vi "CE Center - VC manager.vi"(5 "cmd":enum16{"open", "close", "close all"}(ring)=enum."close", 6 "error in":errorcluster, 9 "VC Handle":T2=-1) -> (0 "error out":errorcluster, 1 "err code":T1 items=["No error", "Invalid variable type", "Variable not found", "Variable already exists", "Invalid context handle", "Input error", "Invalid data format", "No history attached", "History already attached", "Invalid history parameters", "Wrong variable name", "Wrong alias name", "Non-unique alias", "Alias not found", "No alias associated", "Alias already associated", "Wrong context name", "Non-unique context name", "Context name not found", "Invalid parameter", "Generic error", "Unknown error code"], 3 "VC Handle out":T2=-1)   [LabVIEW 2021]
doc: "::: CalcExpress Toolkit :::\nCopyright (c) 2000-2026 Konstantin Shifershteyn. All rights reserved."
uses:
  vi.lib/addons/CalcExpress/cetypes.llb/VarMan Variable Context Handle.ctl
  vi.lib/addons/CalcExpress/cetypes.llb/VarMan Error Code.ctl
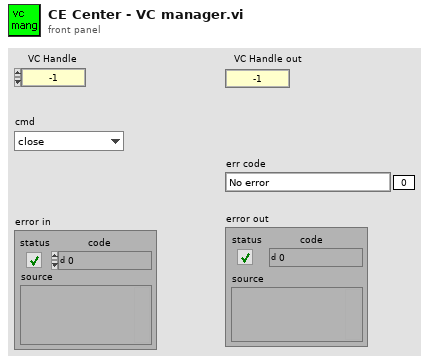
[diagram p1: front panel]
types:
  T1 = typedef "VarMan Error Code.ctl" = u16
  T2 = typedef "VarMan Variable Context Handle.ctl" = i32
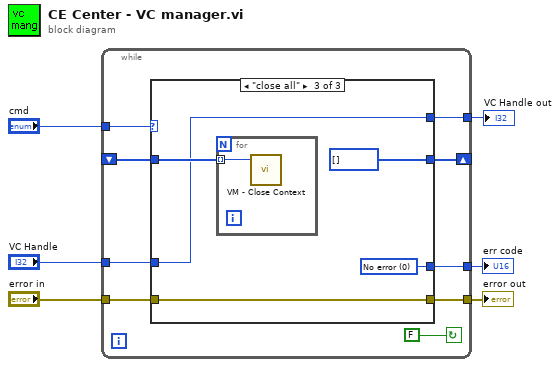
[diagram p0: block diagram]
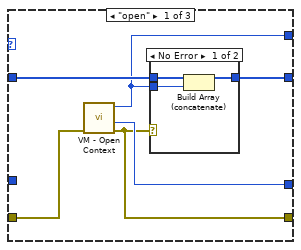
[diagram p2: hidden frame]
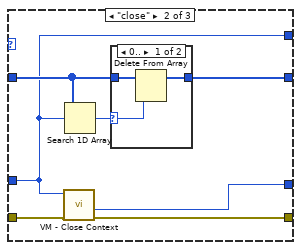
[diagram p4: hidden frame]
diagram:
  n1 = while {
    tunnel: [w8] -> w1
    tunnel: "VC Handle" -> [w9]
    tunnel: "error in" -> [w10]
    tunnel: [w11] -> w4
    tunnel: [w12] -> w5
    tunnel: "cmd" -> [w15]
    shift-left: _ -> [w14]
    shift-right: [w13] -> _
    stop <- FALSE continue-if-true
    n2 = case shown="\"close all\"" w15 {
      tunnel: w14 -> [w21 w32 w40]
      tunnel: [w20 w31 i32[] []] -> w13
      tunnel: [w19 w29 w37] -> w12
      tunnel: [w18 w30 w41] -> w11
      tunnel: w10 -> [w16 w28 w41]
      tunnel: w9 -> [_ w27 w38]
      tunnel: [w17 w27 w38] -> w8
      frame "open" {
        n3 = call "VM - Open Context.vi"("error in"=w16) -> ("error out"=w18:errorcluster, "err code"=w19:T1, "VC Handle out"=w17:T2)  [unwired: 8 in]
        n4 = case shown="No Error" w18 {
          tunnel: w21 -> [w24 w25]
          tunnel: w17 -> [w23 _]
          tunnel: [w22 w25] -> w20
          frame No Error {
            n5 = Build Array (concatenate)(w24, w23) -> (w22:T2[])
          }
          frame Error {
          }
        }
      }
      frame "close" {
        n6 = call "VM - Close Context.vi"("error in"=w28, "VC Handle"=w27) -> ("error out"=w30:errorcluster, "err code"=w29:T1)  [unwired: 8 in]
        n7 = Search 1D Array(1D array=w32, element=w27) -> (index of element=w26:i32)  [unwired: 1 in]
        n8 = case shown="0.." w26 {
          selector: w26 -> [w33 _]
          tunnel: w32 -> [w35 w36]
          tunnel: [w34 w36] -> w31
          frame 0.. {
            n9 = Delete From Array(array=w35, index=w33) -> (array with subset deleted=w34:T2[])  [unwired: 1 in, 1 out]
          }
          frame ..-1 {
          }
        }
      }
      frame "close all" {
        w37 = T1 0 items=["No error", "Invalid variable type", "Variable not found", "Variable already exists", "Invalid context handle", "Input error", "Invalid data format", "No history attached", "History already attached", "Invalid history parameters", "Wrong variable name", "Wrong alias name", "Non-unique alias", "Alias not found", "No alias associated", "Alias already associated", "Wrong context name", "Non-unique context name", "Context name not found", "Invalid parameter", "Generic error", "Memory Full", "Unrecognized LV error", "Unknown error code"] ("err code")
        n10 = for {
          tunnel: w40 -> [w42] mode=indexing
          n11 = call "VM - Close Context.vi"("VC Handle"=w42) -> ()  [unwired: 9 in, 2 out]
        }
      }
    }
  }
  "VC Handle out" <- w1
  "error out" <- w4
  "err code" <- w5
